vi "RT_PROFINET_Adapter.vi"(8 "error in (no error)":errorcluster={"status"=FALSE, "code"=0, "source"="\"\""}, 11 "I/O map and interface refs":string) -> (0 "error out":errorcluster={"status"=FALSE, "code"=0, "source"="\"\""}, 2 "status ok":bool, 3 "I/O image":string)   [LabVIEW 2026]
doc: "INTENT: Exchange PROFINET process I/O through supported hardware. LOGIC: Read/write prevalidated cyclic process data via actual commissioned interface; decode validity bits."
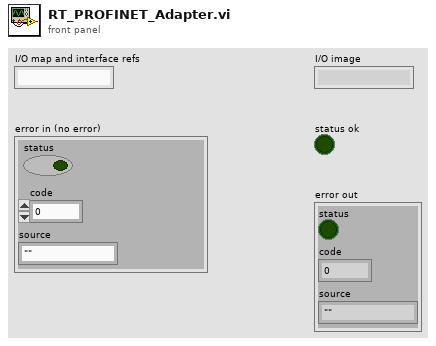
[diagram p1: front panel]
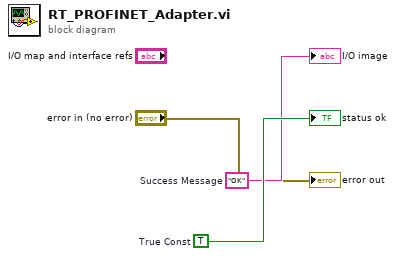
[diagram p0: block diagram]
diagram:
  w3 = TRUE  # True Const
  w2 = "OK"  # Success Message
  "I/O image" <- w2
  "status ok" <- w3
  "error out" <- "error in (no error)"
